vi "Measurement Logic.vi"(8 "error in":errorcluster, 9 "Meas Config":T2={"Input Terminal Name"="Lorem ipsum dolor sit", "Counter Interface"="", "Active Edge"=1, "Pulses"=32, "Timeout (s)"=64, "FD Baudrate"=4294967264, "Baudrate"=4294967264, "FD ISO Mode"=enum."ISO", "IO Mode"=enum."CAN", "CAN Interface Name"="", "Termination CAN"=TRUE, "IDENTIFIER"=1, "PAYLOAD"=[3, 6], "TYPE"=0} {"TYPE" items=["CAN Data"=0, "CAN Remote"=1, "CAN Bus Error"=2, "CAN 2.0 Data"=8, "CAN FD Data"=16, "CAN FD+BRS Data"=24, "J1939 Data"=192, "Delay"=224, "Log Trigger"=225, "Start Trigger"=226]; "PAYLOAD" format="%x"; "IDENTIFIER" format="%x"; "Baudrate" format="%x"; "FD Baudrate" format="%x"; "Active Edge" items=["Rising"=10280, "Falling"=10171]}, 10 "measure call context in":refnum<class "Measure Call Context.lvclass">) -> (0 "error out":errorcluster, 1 "measurement results":T1, 2 "measure call context out":refnum<class "Measure Call Context.lvclass">)   [LabVIEW 2025, in "Workflow DO.lvclass"]
doc: "Contains the core logic for executing the measurement."
uses:
  Workflow DO.lvclass
  <vilib>/Plug-In SDKs/Measurements/Measure Call Context/Measure Call Context.lvclass
  Measurement Configuration.ctl
  Measurement Results.ctl
  <vilib>/DAQmx/read.llb/DAQmx Read (Digital 1D Bool 1Chan 1Samp).vi
  <vilib>/DAQmx/read.llb/DAQmx Read (Counter U32 1Chan 1Samp).vi
  <vilib>/xnet/xnet.llb/XNET Read (Frame CAN).vi
  <vilib>/DAQmx/miscellaneous.llb/DAQmx Fill In Error Info.vi
  <extravilib>/ChannelInstances/Event Messenger-bool/Instantiate.vi
  Workflow DO.lvclass/Workflow DO.ctl
panel:
  out "stop":bool
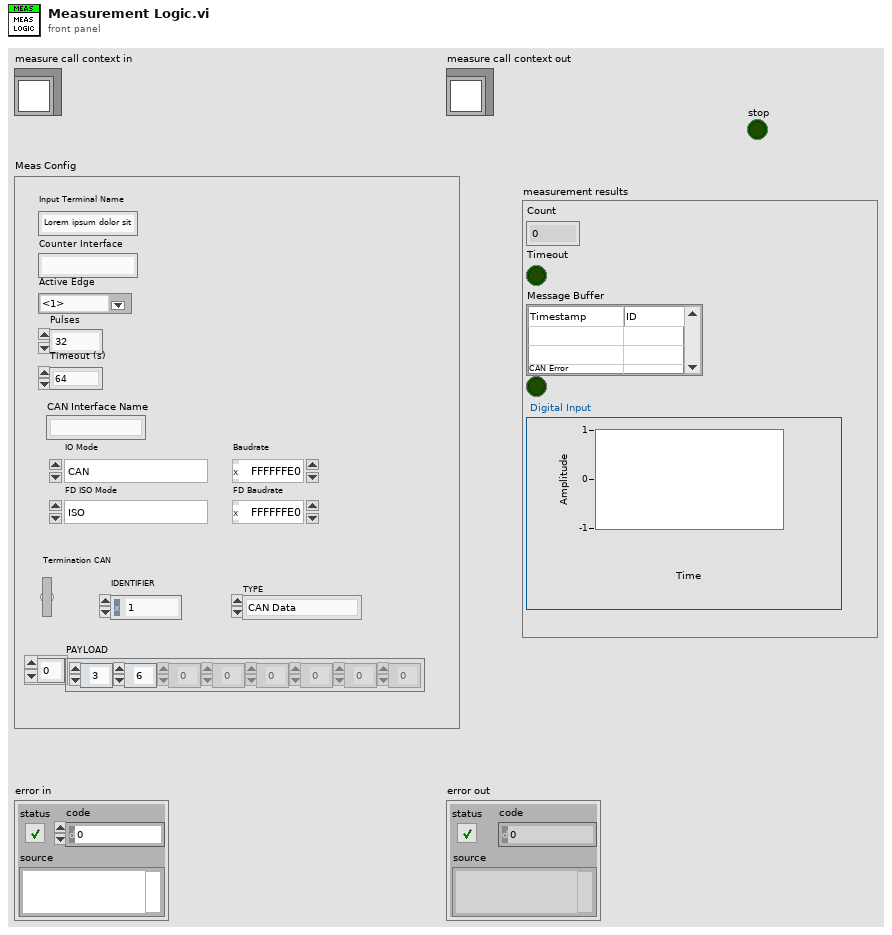
[diagram p1: front panel]
types:
  T1 = typedef "Workflow DO.lvclass/Measurement Results.ctl" = cluster{"Count":u32, "Timeout":bool, "Message Buffer":string[][], "CAN Error":bool, "Digital Input":u32[]}
  T2 = typedef "Workflow DO.lvclass/Measurement Configuration.ctl" = cluster{"Input Terminal Name":string, "Counter Interface":string, "Active Edge":i32, "Pulses":u32, "Timeout (s)":u32, "FD Baudrate":u32, "Baudrate":u32, "FD ISO Mode":enum32{"ISO", "Legacy ISO", "Non-ISO"}, "IO Mode":enum32{"CAN", "CAN FD", "CAN FD + BRS"}, "CAN Interface Name":string, "Termination CAN":bool, "IDENTIFIER":u32, "PAYLOAD":u32[], "TYPE":u32}
  T3 = typedef "XNET Frame CAN.ctl" = cluster{"timestamp":timestamp, "payload":u8[], "identifier":u32, "type":T4, "extended?":bool, "echo?":bool}
  T4 = typedef "XNET Frame Type CAN.ctl" = u8
  T5 = typedef "Event Messenger-bool.lvlib/))Channel.ctl" = refnum<queue>
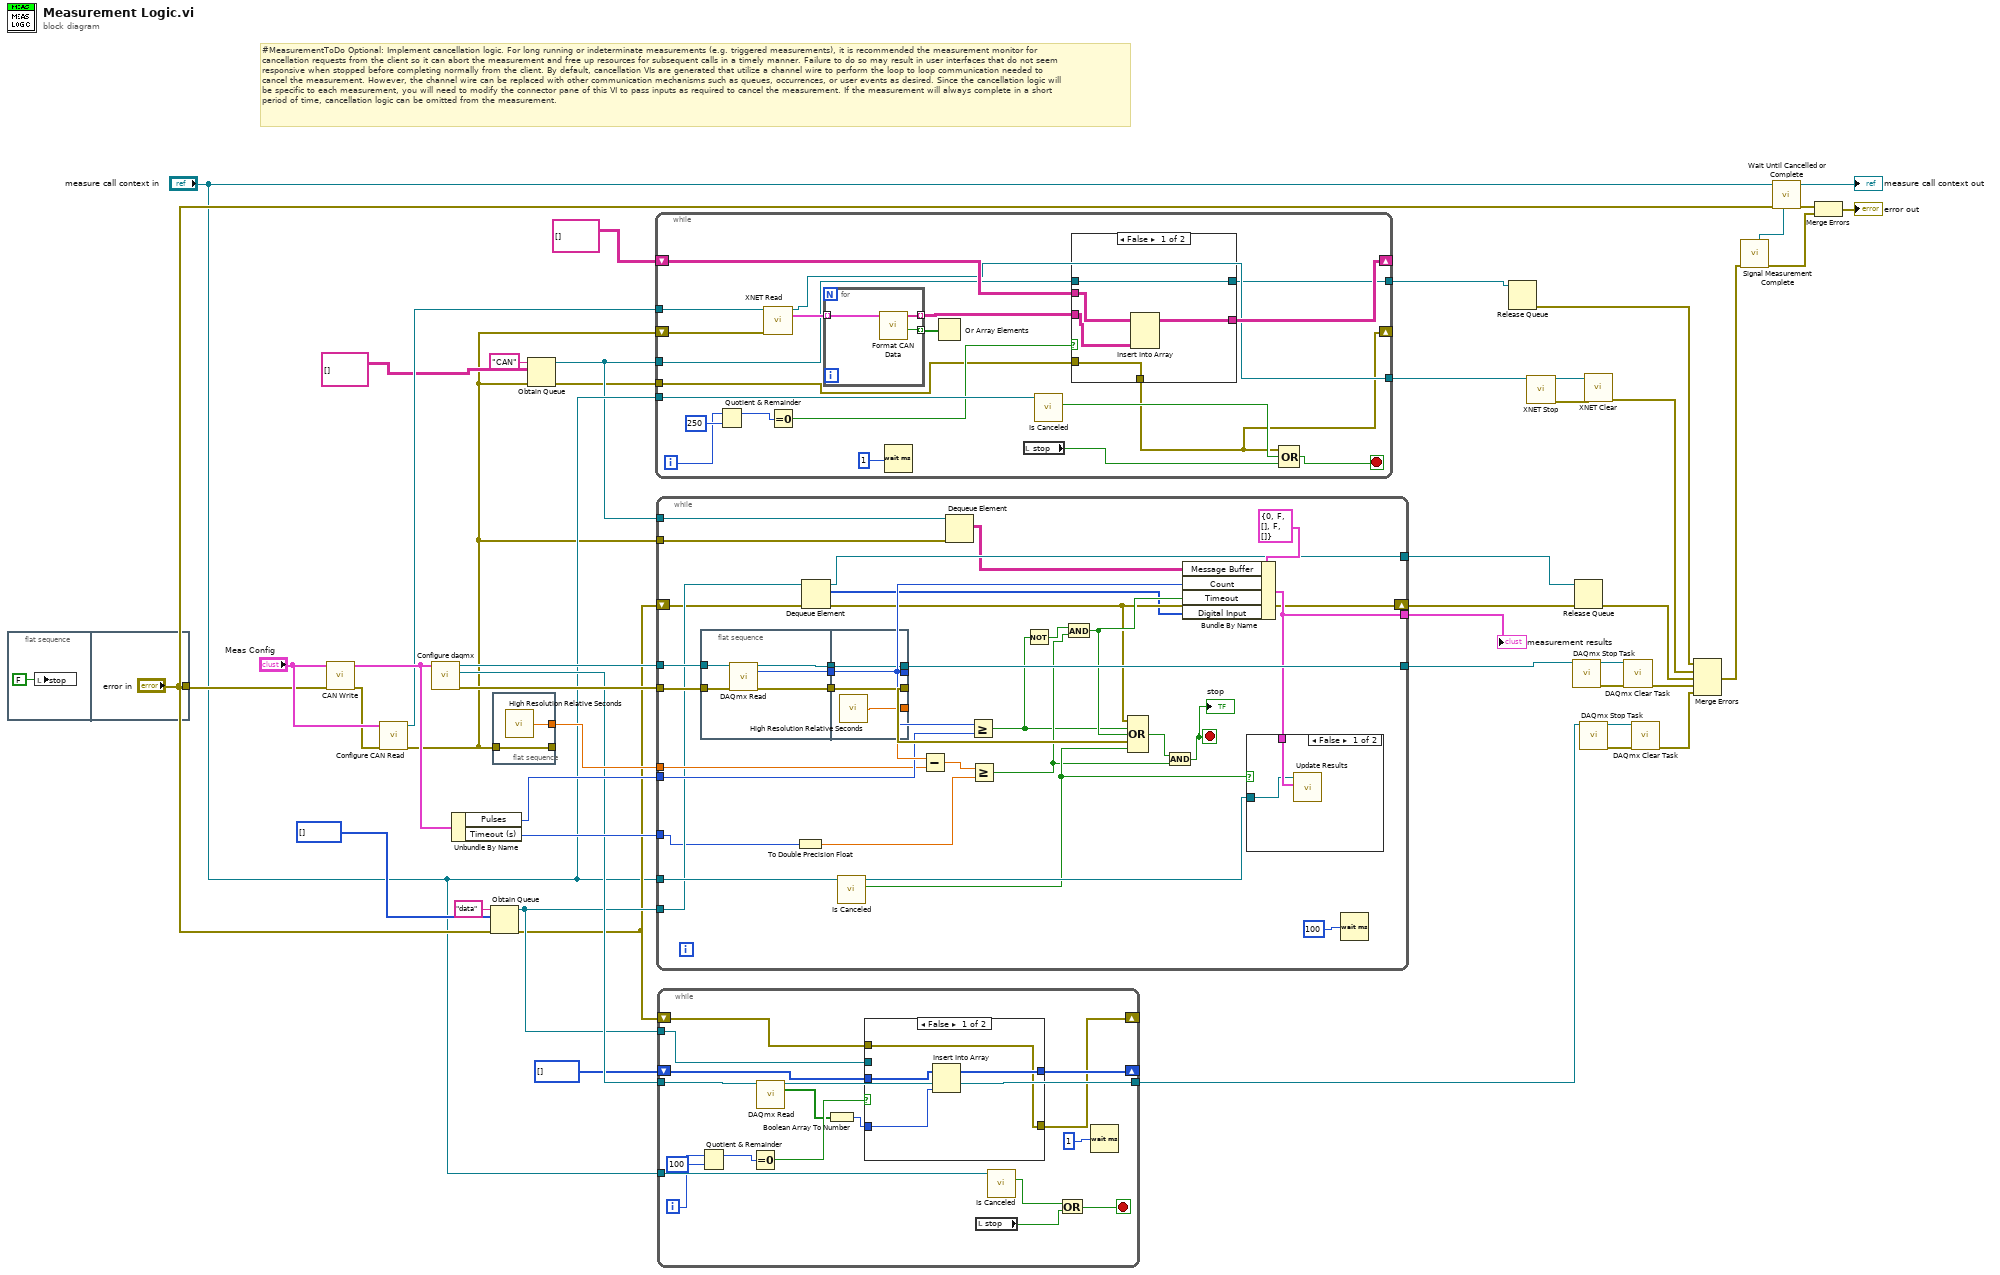
[diagram p0: block diagram]
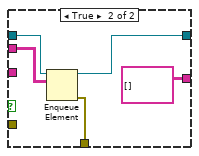
[diagram p2: hidden frame]
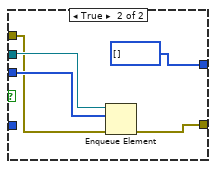
[diagram p3: hidden frame]
diagram:
  # "#MeasurementToDo Optional: Implement cancellation logic. For long running or indeterminate measurements (e.g. triggered measurements), it is recommended the measurement monitor for cancellation requests from the client so it can abort the measurement and free up resources for subsequent calls in a timely manner. Failure to do so may result in user interfaces that do not seem responsive when stopped before completing normally from the client. By default, cancellation VIs are generated that utilize a channel wire to perform the loop to loop communication needed to cancel the measurement. However, the channel wire can be replaced with other communication mechanisms such as queues, occurrences, or user events as desired. Since the cancellation logic will be specific to each measurement, you will need to modify the connector pane of this VI to pass inputs as required to cancel the measurement. If the measurement will always complete in a short period of time, cancellation logic can be omitted from the measurement."
  n1 = flat-sequence {
    tunnel: ["error in"] -> w23
    frame #0 {
      n2 = local write "stop"(FALSE ("stop")) -> ()
    }
    frame #1 {
    }
  }
  n3 = call "CAN Write.vi"("error in"=w23, "Meas Config"="Meas Config") -> ("error out"=w32:errorcluster, "Meas Config"=w38:T2)  [unwired: 7 in, 1 out]
  n4 = call "Configure CAN Read.vi"("error in"=w32, "measurement configuration"="Meas Config") -> ("error out"=w3:errorcluster, "XNET Read"=w12:refnum<k21>)  [unwired: 8 in]
  n5 = call "Configure daqmx.vi"("measurement configuration"=w38) -> ("error out"=w30:errorcluster, "Task out DI"=w22:refnum<k21>, "Task out"=w36:refnum<k21>)  [unwired: 8 in]
  n6 = Unbundle By Name(w38) -> ("Pulses"=w35:u32, "Timeout (s)"=w37:u32)
  n7 = Obtain Queue(name (unnamed)="data", element data type=u32[] [], error in (no error)=w23) -> (queue out=w20:refnum<queue>, error out=w17:errorcluster)  [unwired: 2 in, 1 out]
  n8 = flat-sequence {
    tunnel: [w51] -> w31
    tunnel: w3 -> [w50]
    tunnel: [w50] -> _
    frame #0 {
      n9 = call <vilib>:"High Resolution Relative Seconds.vi"() -> ("relative seconds"=w51:dbl)
    }
  }
  n10 = Obtain Queue(name (unnamed)="CAN", element data type=string[][] [] ("Display"), error in (no error)=w3) -> (queue out=w9:refnum<queue>, error out=w2:errorcluster)  [unwired: 2 in, 1 out]
  n11 = while {
    tunnel: w12 -> [w70]
    tunnel: "measure call context in" -> [w66]
    shift-right: [w57] -> _
    shift-left: string[][] [] ("Display") -> [w59]
    tunnel: w9 -> [w58]
    tunnel: [w55] -> w6
    tunnel: [w54] -> w4
    shift-right: [w52] -> _
    shift-left: w3 -> [w69]
    tunnel: w2 -> [w53]
    i -> [w61]
    stop <- w67 stop-if-true
    n12 = Quotient & Remainder(x=w61, y=250) -> (x-y*floor(x/y)=w62:i32)  [unwired: 1 out]
    n13 = call-poly <vilib>:"XNET Read.vi"("session in"=w70, "error in (no error)"=w69) -> ("session out"=w55:refnum<k21>, "data"=w72:T3[])  [unwired: 10 in, 2 out]
    n14 = Equal To 0?(x=w62) -> (x = 0?=w60:bool)
    n15 = for {
      tunnel: w72 -> [w84] mode=indexing
      tunnel: [w85] -> w56 mode=indexing
      tunnel: [w83] -> w71 mode=indexing
      n16 = call "Format CAN Data.vi"("Frame"=w84) -> ("Error"=w83:bool, "Display"=w85:string[])  [unwired: 8 in, 1 out]
    }
    n17 = Wait (ms)(milliseconds to wait=u32 1 ("Loop Time (ms)")) -> ()  [unwired: 1 out]
    n18 = Or Array Elements(Boolean array=w71) -> ()  [unwired: 1 out]
    n19 = local read "stop"() -> (w68:bool)
    n20 = call <vilib>:"Is Canceled.vi"("measure call context in"=w66) -> ("is canceled?"=w65:bool)  [unwired: 8 in, 2 out]
    n21 = case shown="False" w60 {
      tunnel: w59 -> [w77 w80]
      tunnel: w58 -> [w74 w82]
      tunnel: [w76 string[][] [] ("Display")] -> w57
      tunnel: w56 -> [w75 _]
      tunnel: [w74 w79] -> w54
      tunnel: [w73 w78] -> w52
      tunnel: w53 -> [w73 _]
      frame False {
        n22 = Insert Into Array(array=w77, new element=w75) -> (w76:string[][])  [unwired: 2 in]
      }
      frame True {
        n23 = Enqueue Element(queue=w82, element=w80) -> (queue out=w79:refnum<queue>, error out=w78:errorcluster)  [unwired: 2 in, 1 out]
      }
    }
    n24 = Compound Arithmetic op=OR(w52, w65, w68) -> (w67:bool)
  }
  n25 = while {
    tunnel: "measure call context in" -> [w117]
    tunnel: w36 -> [w109]
    tunnel: [w119] -> w40
    tunnel: w37 -> [w95]
    tunnel: w35 -> [w110]
    tunnel: w31 -> [w108]
    tunnel: w30 -> [w107]
    tunnel: [w105] -> w28
    tunnel: w20 -> [w103]
    shift-right: [w99] -> w16
    shift-left: w17 -> [w97]
    tunnel: [w98] -> w15
    tunnel: w9 -> [w88]
    tunnel: w3 -> [w86]
    stop <- w91 stop-if-true
    n26 = flat-sequence {
      tunnel: [w124] -> w115
      tunnel: [w120] -> w114
      tunnel: [w123] -> w113
      tunnel: w109 -> [w122]
      tunnel: w107 -> [w121]
      tunnel: [w126] -> w116
      tunnel: [w127] -> w111
      tunnel: [w128] -> w119
      tunnel: w115 -> [w128]
      tunnel: w114 -> [w127]
      tunnel: w113 -> [w126]
      tunnel: [w125] -> w112
      frame #0 {
        n27 = call-poly <vilib>:"DAQmx Read.vi"("task/channels in"=w122, "error in"=w121) -> ("task out"=w124:refnum<k21>, "data"=w120:u32, "error out"=w123:errorcluster)  [unwired: 11 in]
      }
      frame #1 {
        n28 = call <vilib>:"High Resolution Relative Seconds.vi"() -> ("relative seconds"=w125:dbl)
      }
    }
    n29 = To Double Precision Float(number=w95) -> (double precision float=w94:dbl)
    n30 = Dequeue Element(queue=w103, error in (no error)=w97) -> (queue out=w98:refnum<queue>, element=w89:u32[], error out=w99:errorcluster)  [unwired: 1 in, 1 out]
    n31 = call <vilib>:"Is Canceled.vi"("measure call context in"=w117) -> ("is canceled?"=w102:bool, "measure call context out"=w104:refnum<class "Measure Call Context.lvclass">)  [unwired: 8 in, 1 out]
    n32 = Subtract(x=w112, y=w108) -> (x-y=w93:dbl)
    n33 = Dequeue Element(queue=w88, error in (no error)=w86) -> (element=w87:string[][])  [unwired: 1 in, 3 out]
    n34 = Greater Or Equal?(x=w111, y=w110) -> (x >= y?=w90:bool)
    n35 = Greater Or Equal?(x=w93, y=w94) -> (x >= y?=w96:bool)
    n36 = Not(x=w90) -> (.not. x?=w101:bool)
    n37 = And(x=w101, y=w96) -> (x .and. y?=w100:bool)
    n38 = Compound Arithmetic op=OR(w99, w90, w100, w116, w102) -> (w92:bool)
    n39 = And(x=w92, y=w96) -> (x .and. y?=w91:bool)
    "stop" <- w91
    n40 = Bundle By Name(cluster=T1 {"Count"=0, "Timeout"=FALSE, "Message Buffer"=[], "CAN Error"=FALSE, "Digital Input"=[]} ("measurement results"), "Message Buffer"=w87, "Count"=w111, "Timeout"=w100, "Digital Input"=w89) -> (w105:T1)
    n41 = case shown="False" w102 {
      tunnel: w105 -> [w130 _]
      tunnel: w104 -> [w129 _]
      frame False {
        n42 = call <vilib>:"Update Results.vi"("measurement results"=w130, "measure call context in"=w129) -> ()  [unwired: 8 in, 2 out]
      }
      frame True {
      }
    }
    n43 = Wait (ms)(milliseconds to wait=u32 100 ("Loop Time (ms)")) -> ()  [unwired: 1 out]
  }
  "measurement results" <- w28
  n44 = while {
    tunnel: "measure call context in" -> [w147]
    tunnel: [w146] -> w24
    tunnel: w20 -> [w145]
    tunnel: w22 -> [w144]
    shift-right: [w136] -> _
    shift-left: u32[] [] -> [w135]
    shift-right: [w131] -> _
    shift-left: w17 -> [w132]
    i -> [w142]
    stop <- w134 stop-if-true
    n45 = Quotient & Remainder(x=w142, y=100) -> (x-y*floor(x/y)=w140:i32)  [unwired: 1 out]
    n46 = Equal To 0?(x=w140) -> (x = 0?=w139:bool)
    n47 = call-poly <vilib>:"DAQmx Read.vi"("task/channels in"=w144) -> ("task out"=w146:refnum<k21>, "data"=w138:bool[])  [unwired: 12 in, 1 out]
    n48 = Boolean Array To Number(Boolean array=w138) -> (number=w137:u32)
    n49 = case shown="False" w139 {
      tunnel: w145 -> [_ w157]
      tunnel: w137 -> [w151 _]
      tunnel: w135 -> [w152 w156]
      tunnel: [w150 u32[] []] -> w136
      tunnel: w132 -> [w149 w154]
      tunnel: [w149 w153] -> w131
      frame False {
        n50 = Insert Into Array(array=w152, new element=w151) -> (w150:u32[])  [unwired: 1 in]
      }
      frame True {
        n51 = Enqueue Element(queue=w157, element=w156, error in (no error)=w154) -> (error out=w153:errorcluster)  [unwired: 1 in, 2 out]
      }
    }
    n52 = local read "stop"() -> (w133:bool)
    n53 = call <vilib>:"Is Canceled.vi"("measure call context in"=w147) -> ("is canceled?"=w148:bool)  [unwired: 8 in, 2 out]
    n54 = Or(x=w148, y=w133) -> (x .or. y?=w134:bool)
    n55 = Wait (ms)(milliseconds to wait=u32 1 ("Loop Time (ms)")) -> ()  [unwired: 1 out]
  }
  n56 = Release Queue(queue=w4) -> (error out=w1:errorcluster)  [unwired: 2 in, 2 out]
  n57 = call <vilib>:"XNET Stop.vi"("session in"=w6) -> ("session out"=w29:refnum<k21>, "error out"=w5:errorcluster)  [unwired: 13 in]
  n58 = call <vilib>:"DAQmx Stop Task.vi"("task/channels in"=w40) -> ("task out"=w41:refnum<k21>, "error out"=w42:errorcluster)  [unwired: 13 in]
  n59 = Release Queue(queue=w15, error in (no error)=w16) -> (error out=w14:errorcluster)  [unwired: 1 in, 2 out]
  n60 = call <vilib>:"DAQmx Stop Task.vi"("task/channels in"=w24) -> ("task out"=w25:refnum<k21>, "error out"=w27:errorcluster)  [unwired: 13 in]
  n61 = call <vilib>:"XNET Clear.vi"("session in"=w29, "error in (no error)"=w5) -> ("error out"=w13:errorcluster)  [unwired: 13 in]
  n62 = call <vilib>:"DAQmx Clear Task.vi"("task in"=w41, "error in"=w42) -> ("error out"=w39:errorcluster)  [unwired: 13 in]
  n63 = call <vilib>:"DAQmx Clear Task.vi"("task in"=w25, "error in"=w27) -> ("error out"=w26:errorcluster)  [unwired: 13 in]
  n64 = Merge Errors(w1, w13, w14, w39, w26) -> (w33:errorcluster)
  n65 = call "Signal Measurement Complete.vi"("error in (no error)"=w33) -> ("error out"=w45:errorcluster, "done channel"=w46:T5)  [unwired: 9 in]
  n66 = call "Wait Until Cancelled or Complete.vi"("done channel"=w46, "error in (no error)"=w23, "measure call context in"="measure call context in") -> ("error out"=w44:errorcluster, "measure call context out"=→"measure call context out":refnum<class "Measure Call Context.lvclass">)  [unwired: 7 in]
  n67 = Merge Errors(w44, w45) -> (→"error out":errorcluster)
